vi "CIF Get Subscriber Stats.vi"(8 "error in (no error)":errorcluster, 11 "Subscriber Reference":T2 {"refnum" format="%.0x"}) -> (0 "error out":errorcluster, 2 "Last Cnt":u64, 3 "CIF Subscriber Stats":T1)   [LabVIEW 2021, in "Iceoryx.lvlib"]
uses:
  Iceoryx.lvlib
  typedef/CIF Pcap Subscriber Stats.ctl
  SubVIs/Convert Error Core.vi
  Refnum/Typedef/CIF Subscriber Refnum.ctl
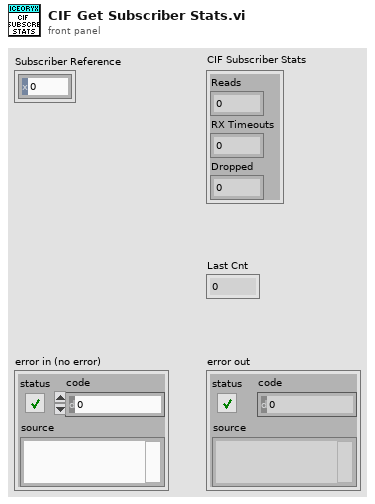
[diagram p1: front panel]
types:
  T1 = typedef "Iceoryx.lvlib/CIF Pcap Subscriber Stats.ctl" = cluster{"Reads":u64, "RX Timeouts":u64, "Dropped":u64}
  T2 = typedef "Iceoryx.lvlib/CIF Subscriber Refnum.ctl" = cluster{"refnum":u64, "CIF Sub":enum8{"cifsub"}}
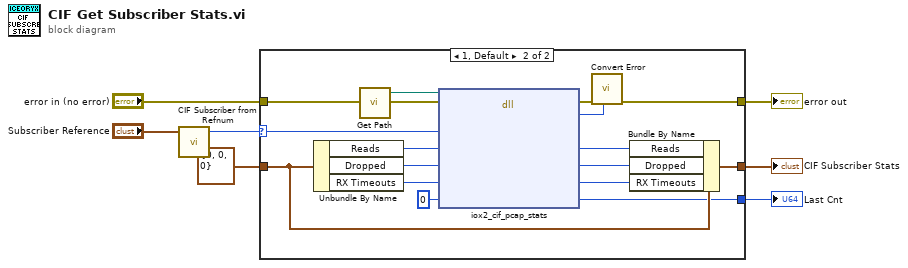
[diagram p0: block diagram]
diagram:
  n1 = call "CIF Subscriber from Refnum.vi"("CIF Subscriber Refnum"="Subscriber Reference") -> ("CIF Subscriber U64"=w1:u64)  [unwired: 4 in]
  n2 = case shown="1, Default" w1 {
    selector: w1 -> [_ w20]
    tunnel: "error in (no error)" -> [w9 w25]
    tunnel: [w9 w21] -> w6
    tunnel: T1 {"Reads"=0, "RX Timeouts"=0, "Dropped"=0} ("CIF Subscriber Stats") -> [w8 w16]
    tunnel: [w8 w12] -> w3
    tunnel: [_ w10] -> w2
    frame 0 {
    }
    frame 1, Default {
      n3 = Unbundle By Name(w16) -> ("Reads"=w19:u64, "Dropped"=w17:u64, "RX Timeouts"=w18:u64)
      n4 = call "Get Path.vi"() -> ("libiox2_cif path"=w24:path)  [unwired: 4 in]
      n5 = dll-call lib="D:/dev/iceoryx2_lvwrapper/dist/iox2_cif.dll" fn="iox2_cif_pcap_stats"(path in=w24, error in=w25, "subscriber"=w20, "samples"=w19, "dropped"=w17, "timeouts"=w18, "last_ctr"=u64 0) -> (error out=w23:errorcluster, "return type"=w22:i32, "samples"=w15:u64, "dropped"=w13:u64, "timeouts"=w14:u64, "last_ctr"=w10:u64)  [unwired: 2 in, 1 out]
      n6 = call "Convert Error.vi"("return type"=w22, "error in (no error)"=w23) -> ("error out"=w21:errorcluster)  [unwired: 9 in]
      n7 = Bundle By Name(cluster=w16, "Reads"=w15, "Dropped"=w13, "RX Timeouts"=w14) -> (w12:T1)
    }
  }
  "error out" <- w6
  "CIF Subscriber Stats" <- w3
  "Last Cnt" <- w2
